vi "Example_Table_Append.vi"(9 "max rows":i32=50, 10 "rows":string[][](array[string]), 11 "table in":string[][](array[string])) -> (3 "table out":string[][](array[string]))   [LabVIEW 2021]
doc: "Example: appends rows to a display table and keeps the newest max rows."
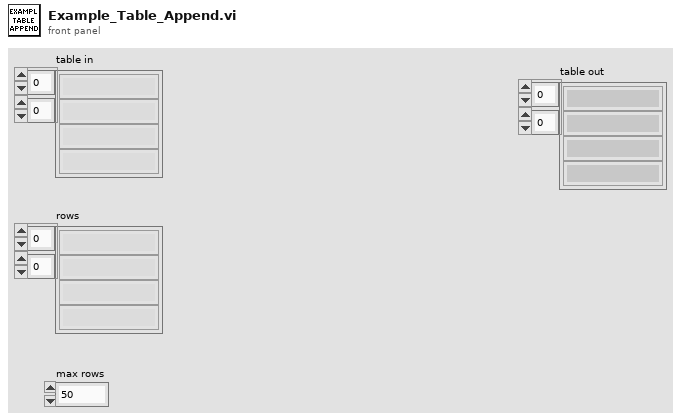
[diagram p1: front panel]
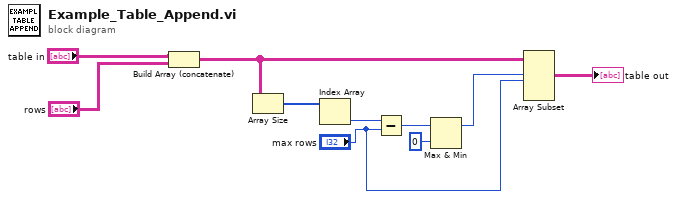
[diagram p0: block diagram]
diagram:
  n1 = Build Array (concatenate)("table in", "rows") -> (w4:string[][])
  n2 = Array Size(array=w4) -> (size(s)=w8:i32[])
  n3 = Index Array(array=w8) -> (element=w7:i32)  [unwired: 1 in]
  n4 = Subtract(x=w7, y="max rows") -> (x-y=w6:i32)
  n5 = Max & Min(x=w6, y=0) -> (max(x,y)=w1:i32)  [unwired: 1 out]
  n6 = Array Subset(array=w4, index (row)=w1, length (row)="max rows") -> (→"table out":string[][])  [unwired: 2 in]
